vi "Check Setpoint.vi"(0 "Positions":dbl[](array[numeric]), 2 "Actions":T1, 7 "Limits":dbl[][](array[numeric]), 11 "Setpoints":dbl[](array[numeric]), 13 "Use Limits":bool) -> (8 "Setpoints Out":dbl[](array[numeric]))   [LabVIEW 2021]
uses:
  Stages Controls/Stage Actions.ctl
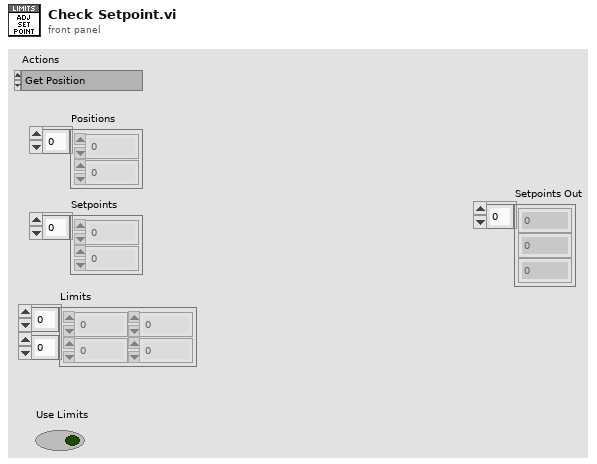
[diagram p1: front panel]
types:
  T1 = typedef "Stage Actions.ctl" = enum16{"Get Position", "SERVO OFF", "SERVO ON", "SERVO ON/OFF", "MVR", "MOVE", "HALT", "ONTARGET", "ERROR", "REFERENCE", "INIT", "VELOCITY", "STATUS", "EXIT", "HOME", "ZEROPOS", "NANOPOS", "ANALOG", "QUIT"}
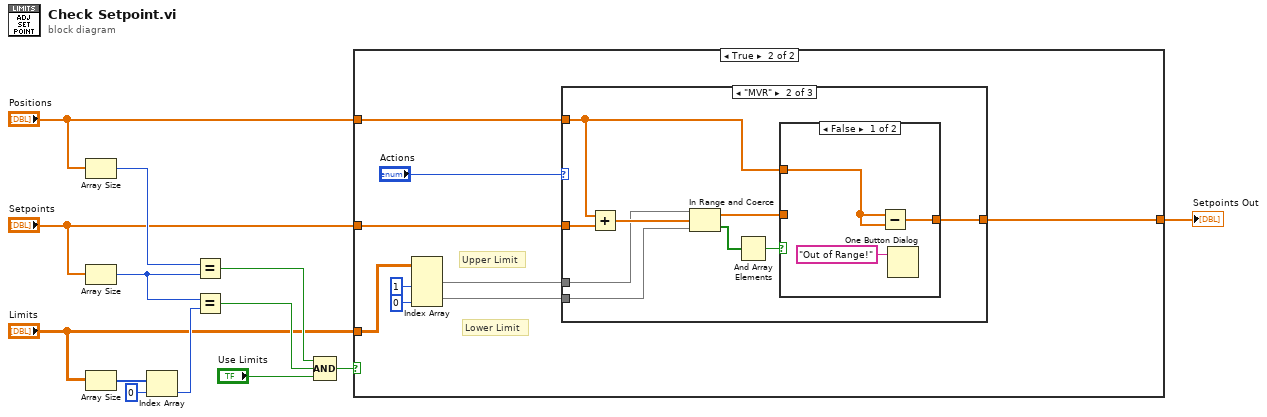
[diagram p0: block diagram]
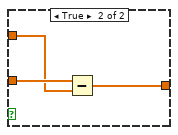
[diagram p4: hidden frame]
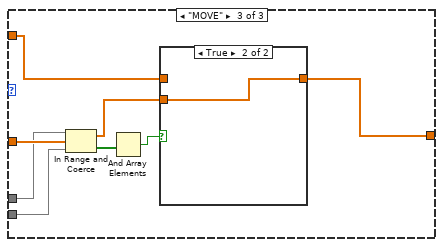
[diagram p5: hidden frame]
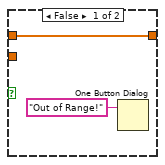
[diagram p6: hidden frame]
diagram:
  n1 = Array Size(array="Positions") -> (size(s)=w11:i32)
  n2 = Array Size(array="Setpoints") -> (size(s)=w9:i32)
  n3 = Array Size(array="Limits") -> (size(s)=w13:i32[])
  n4 = Index Array(array=w13, index=0) -> (element=w10:i32)
  n5 = Equal?(x=w11, y=w9) -> (x = y?=w6:bool)
  n6 = Equal?(x=w9, y=w10) -> (x = y?=w7:bool)
  n7 = Compound Arithmetic op=AND(w6, w7, "Use Limits") -> (w8:bool)
  n8 = case shown="True" w8 {
    tunnel: "Limits" -> [_ w20]
    tunnel: "Setpoints" -> [w14 w22]
    tunnel: "Positions" -> [_ w21]
    tunnel: [w14 w15] -> w1
    frame False {
    }
    frame True {
      # "Upper Limit"
      # "Lower Limit"
      n9 = Index Array(array=w20, index (col) #1=1 ("disabled index (col)"), index (col) #2=0 ("index (col)")) -> (element #1=w17:dbl[], element #2=w16:dbl[])  [unwired: 2 in]
      n10 = case shown="\"MVR\"" "Actions" {
        tunnel: w22 -> [w24 w33 w47]
        tunnel: w21 -> [_ w28 w41]
        tunnel: w17 -> [_ w31 w46]
        tunnel: w16 -> [_ w30 w45]
        tunnel: [w24 w27 w40] -> w15
        frame Default {
        }
        frame "MVR" {
          n11 = Add(x=w28, y=w33) -> (x+y=w32:dbl[])
          n12 = In Range and Coerce(upper limit=w31, x=w32, lower limit=w30) -> (coerced(x)=w29:dbl[], In Range?=w26:bool[])
          n13 = And Array Elements(Boolean array=w26) -> (logical AND=w25:bool)
          n14 = case shown="False" w25 {
            tunnel: w29 -> [_ w39]
            tunnel: w28 -> [w36 w38]
            tunnel: [w35 w37] -> w27
            frame False {
              n15 = Subtract(x=w36, y=w36) -> (x-y=w35:dbl[])
              n16 = One Button Dialog(message="Out of Range!") -> ()  [unwired: 1 in, 1 out]
            }
            frame True {
              n17 = Subtract(x=w39, y=w38) -> (x-y=w37:dbl[])
            }
          }
        }
        frame "MOVE" {
          n18 = In Range and Coerce(upper limit=w46, x=w47, lower limit=w45) -> (coerced(x)=w42:dbl[], In Range?=w44:bool[])
          n19 = And Array Elements(Boolean array=w44) -> (logical AND=w43:bool)
          n20 = case shown="True" w43 {
            tunnel: w42 -> [_ w50]
            tunnel: [w48 w50] -> w40
            tunnel: w41 -> [w48 _]
            frame False {
              n21 = One Button Dialog(message="Out of Range!") -> ()  [unwired: 1 in, 1 out]
            }
            frame True {
            }
          }
        }
      }
    }
  }
  "Setpoints Out" <- w1
